vi "Periodic Tasks.vi"(8 "error in":errorcluster) -> ()   [LabVIEW 2017]
doc: "This VI runs in parallel to other robot code. It can contain as many user-defined periodic loops as you need. These can carry out PID or other sorts of timed response."
uses:
  <vilib>/Rock Robotics/WPI/DriverStation/WPI_DriverStationRobotMode2.ctl
  Robot Global Data.vi
  <vilib>/Rock Robotics/Network Tables/NT Read String.vi
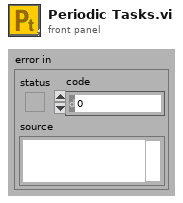
[diagram p1: front panel]
types:
  T1 = typedef "WPI_DriverStationRobotMode2.ctl" = enum16{"Autonomous Disabled", "Autonomous Enabled", "Teleop Disabled", "Teleop Enabled", "Disconnected", "Finish", "Test Disabled", "Test Enabled", "Emergency Stopped"}
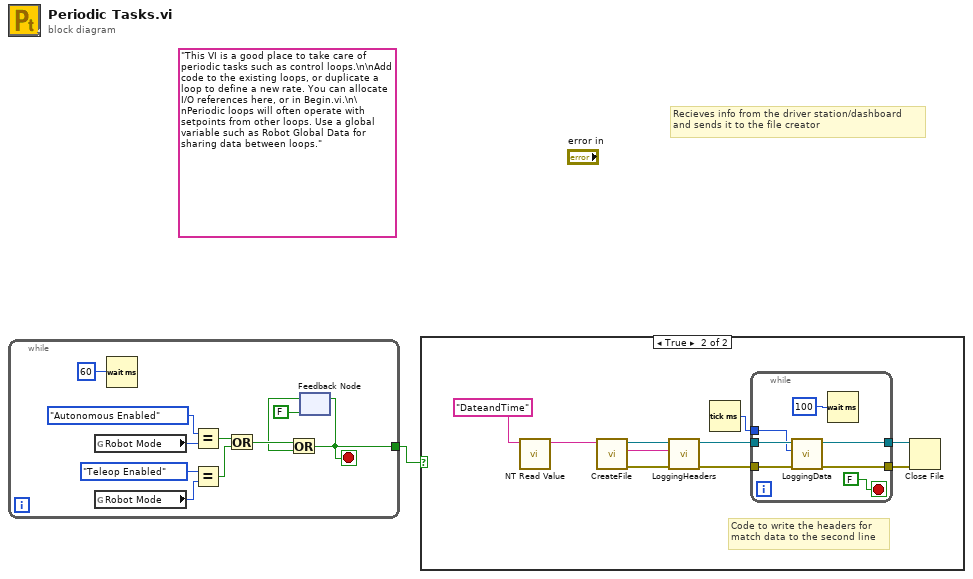
[diagram p0: block diagram]
diagram:
  (unwired) "This VI is a good place to take care of periodic tasks such as control loops.\n\nAdd code to the existing loops, or duplicate a loop to define a new rate. You can allocate I/O references here, or in Begin.vi.\n\nPeriodic loops will often operate with setpoints from other loops. Use a global variable such as Robot Global Data for sharing data between loops."
  # "Recieves info from the driver station/dashboard\nand sends it to the file creator"
  n1 = while {
    tunnel: [w3] -> w1
    stop <- w3 stop-if-true
    n2 = global read "Robot Global Data.vi" "Robot Mode"() -> (w11:T1)
    n3 = global read "Robot Global Data.vi" "Robot Mode"() -> (w10:T1)
    n4 = Wait (ms)(milliseconds to wait=u32 60) -> ()  [unwired: 1 out]
    n5 = Equal?(x=WPI_DriverStationRobotMode2."Autonomous Enabled", y=w11) -> (x = y?=w7:bool)
    n6 = Equal?(x=WPI_DriverStationRobotMode2."Teleop Enabled", y=w10) -> (x = y?=w8:bool)
    n7 = Or(x=w7, y=w8) -> (x .or. y?=w5:bool)
    n8 = feedback #1(FALSE) -> (w4:bool)
    n9 = Or(x=w5, y=w4) -> (x .or. y?=w3:bool)
    n10 = feedback-in #1(w3) -> ()
  }
  n11 = case shown="True" w1 {
    frame False {
    }
    frame True {
      # "Code to write the headers for \nmatch data to the second line"
      n12 = call-poly <vilib>:"NT Read Value.vi"("Name"="DateandTime") -> ("String"=w13:string)  [unwired: 9 in, 1 out]
      n13 = call "CreateFile.vi"("Date/time"=w13) -> ("error out"=w20:errorcluster, "Date/Time"=w22:string, "Byte Stream File out"=w21:refnum<file>)  [unwired: 8 in]
      n14 = call "LoggingHeaders.vi"("error in"=w20, "Date and Time"=w22, "refnum in"=w21) -> ("error out"=w17:errorcluster, "refnum out"=w18:refnum<file>)  [unwired: 7 in]
      n15 = Tick Count (ms)() -> (millisecond timer value=w19:u32)
      n16 = while {
        tunnel: w19 -> [w25]
        tunnel: w18 -> [w27]
        tunnel: w17 -> [w26]
        tunnel: [w24] -> w16
        tunnel: [w23] -> w15
        stop <- FALSE stop-if-true
        n17 = call "LoggingData.vi"("error in (no error)"=w26, "Start time"=w25, "Refmum"=w27) -> ("error out"=w23:errorcluster, "Byte Stream File out"=w24:refnum<file>)  [unwired: 7 in]
        n18 = Wait (ms)(milliseconds to wait=u32 100) -> ()  [unwired: 1 out]
      }
      n19 = Close File(refnum=w16, error in=w15) -> ()  [unwired: 2 out]
    }
  }
